vi "Update Measurement from Metadata.vi"(7 "client service_class":string, 8 "error in":errorcluster, 9 "default value":variant, 10 "metadata":T1, 11 "file refnums":refnum<vi>[](array[refnum])) -> (0 "error out":errorcluster)   [LabVIEW 2021, in "NI Measurement V2 Client Generator Runtime.lvlib"]
uses:
  NI Measurement V2 Client Generator Runtime.lvlib
  <vilib>/gRPC/Generated APIs/ni/measurementlink/measurement/v2/Measurement Service Client V2/RPC Messages/ni_measurementlink_measurement_v2_GetMetadataResponse.ctl
  <vilib>/gRPC/Generated APIs/ni/measurementlink/measurement/v2/Measurement Service Client V2/RPC Messages/ni_measurementlink_measurement_v2_MeasurementDetails.ctl
  <vilib>/gRPC/Generated APIs/ni/measurementlink/measurement/v2/Measurement Service Client V2/RPC Messages/ni_measurementlink_measurement_v2_MeasurementSignature.ctl
  <vilib>/gRPC/Generated APIs/ni/measurementlink/measurement/v2/Measurement Service Client V2/RPC Messages/ni_measurementlink_measurement_v2_ConfigurationParameter.ctl
  <vilib>/gRPC/Generated APIs/ni/measurementlink/measurement/v2/Measurement Service Client V2/RPC Messages/google_protobuf_Field_Kind.ctl
  <vilib>/gRPC/Generated APIs/ni/measurementlink/measurement/v2/Measurement Service Client V2/RPC Messages/ni_measurementlink_measurement_v2_ConfigurationParameter_AnnotationsEntry.ctl
  <vilib>/gRPC/Generated APIs/ni/measurementlink/measurement/v2/Measurement Service Client V2/RPC Messages/google_protobuf_Any.ctl
  <vilib>/gRPC/Generated APIs/ni/measurementlink/measurement/v2/Measurement Service Client V2/RPC Messages/ni_measurementlink_measurement_v2_Output.ctl
  <vilib>/gRPC/Generated APIs/ni/measurementlink/measurement/v2/Measurement Service Client V2/RPC Messages/ni_measurementlink_measurement_v2_Output_AnnotationsEntry.ctl
  <vilib>/gRPC/Generated APIs/ni/measurementlink/measurement/v2/Measurement Service Client V2/RPC Messages/ni_measurementlink_measurement_v2_UserInterfaceDetails.ctl
  <vilib>/Utility/traverseref.llb/TRef TravTarget.ctl
  Client Generator Error Strings Global.vi
  <vilib>/Utility/traverseref.llb/VI Scripting - Traverse.lvlib
  <vilib>/gRPC/Generated APIs/ni/measurementlink/measurement/v2/Measurement Service Client V2/Measurement Service Client V2.lvlib
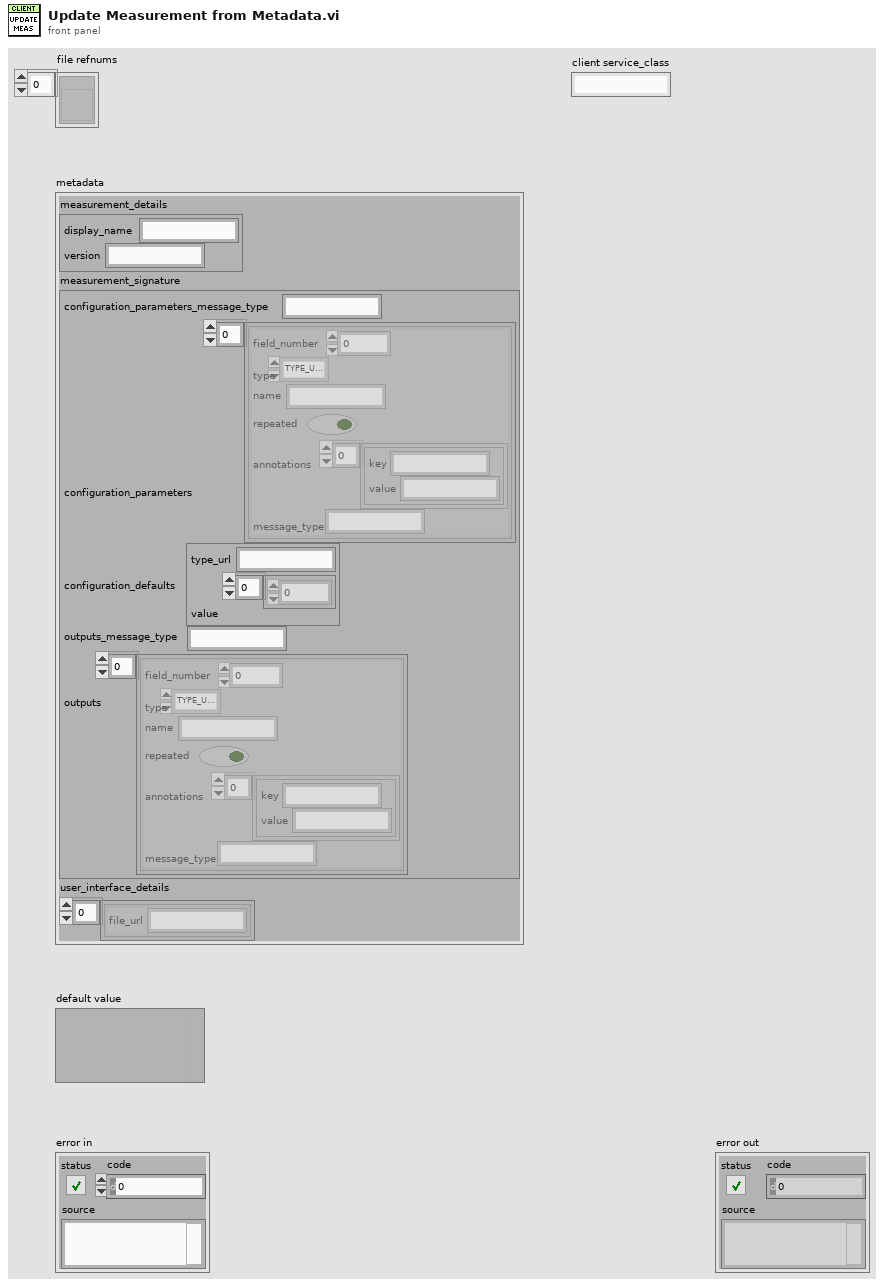
[diagram p1: front panel]
types:
  T1 = typedef "Measurement Service Client V2.lvlib/ni_measurementlink_measurement_v2_GetMetadataResponse.ctl" = cluster{"measurement_details":T2, "measurement_signature":T3, "user_interface_details":T10[]}
  T2 = typedef "Measurement Service Client V2.lvlib/ni_measurementlink_measurement_v2_MeasurementDetails.ctl" = cluster{"display_name":string, "version":string}
  T3 = typedef "Measurement Service Client V2.lvlib/ni_measurementlink_measurement_v2_MeasurementSignature.ctl" = cluster{"configuration_parameters_message_type":string, "configuration_parameters":T4[], "configuration_defaults":T7, "outputs_message_type":string, "outputs":T8[]}
  T4 = typedef "Measurement Service Client V2.lvlib/ni_measurementlink_measurement_v2_ConfigurationParameter.ctl" = cluster{"field_number":i32, "type":T5, "name":string, "repeated":bool, "annotations":T6[], "message_type":string}
  T5 = typedef "Measurement Service Client V2.lvlib/google_protobuf_Field_Kind.ctl" = enum32{"TYPE_UNKNOWN", "TYPE_DOUBLE", "TYPE_FLOAT", "TYPE_INT64", "TYPE_UINT64", "TYPE_INT32", "TYPE_FIXED64", "TYPE_FIXED32", "TYPE_BOOL", "TYPE_STRING", "TYPE_GROUP", "TYPE_MESSAGE", "TYPE_BYTES", "TYPE_UINT32", "TYPE_ENUM", "TYPE_SFIXED32", "TYPE_SFIXED64", "TYPE_SINT32", "TYPE_SINT64"}
  T6 = typedef "Measurement Service Client V2.lvlib/ni_measurementlink_measurement_v2_ConfigurationParameter_AnnotationsEntry.ctl" = cluster{"key":string, "value":string}
  T7 = typedef "Measurement Service Client V2.lvlib/google_protobuf_Any.ctl" = cluster{"type_url":string, "value":u8[]}
  T8 = typedef "Measurement Service Client V2.lvlib/ni_measurementlink_measurement_v2_Output.ctl" = cluster{"field_number":i32, "type":T5, "name":string, "repeated":bool, "annotations":T9[], "message_type":string}
  T9 = typedef "Measurement Service Client V2.lvlib/ni_measurementlink_measurement_v2_Output_AnnotationsEntry.ctl" = cluster{"key":string, "value":string}
  T10 = typedef "Measurement Service Client V2.lvlib/ni_measurementlink_measurement_v2_UserInterfaceDetails.ctl" = cluster{"file_url":string}
  T11 = typedef "TRef TravTarget.ctl" = enum16{"FP", "BD", "Other"}
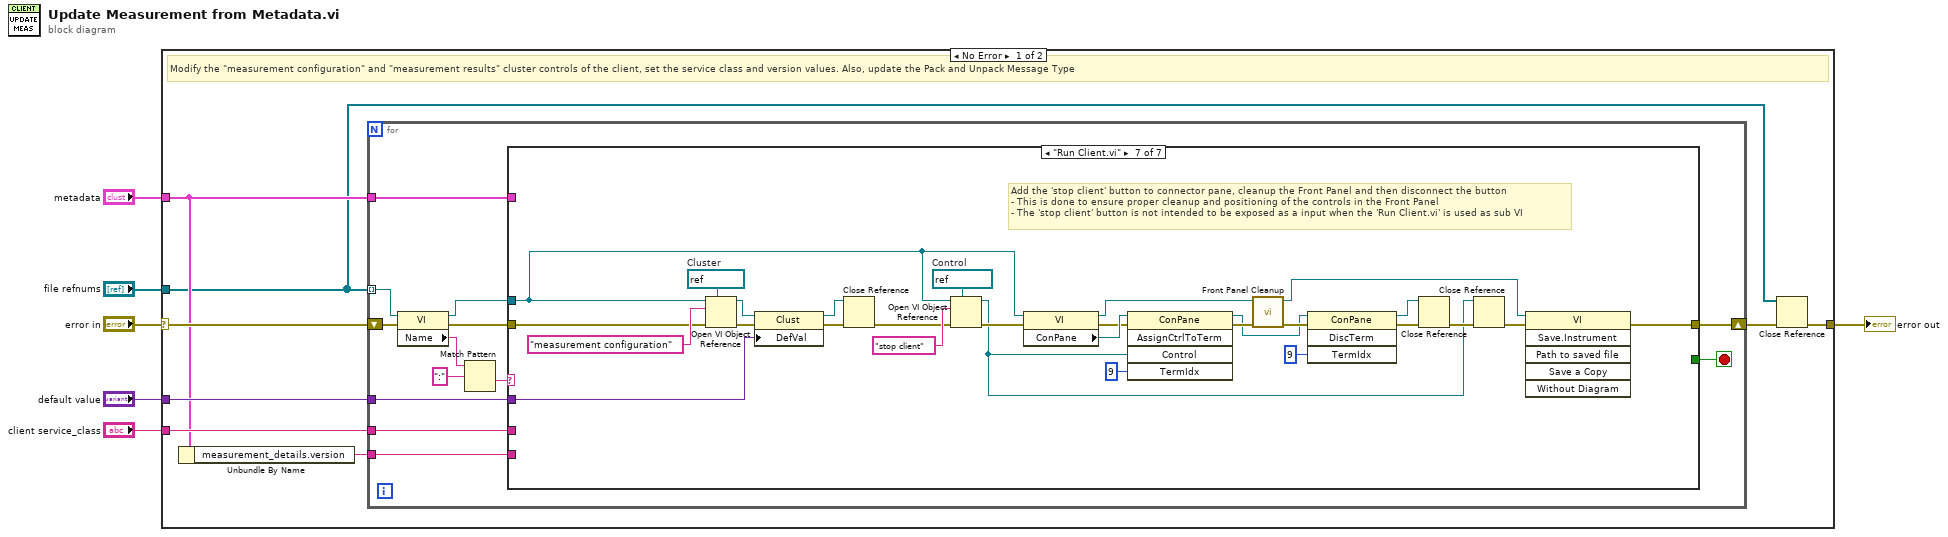
[diagram p0: block diagram]
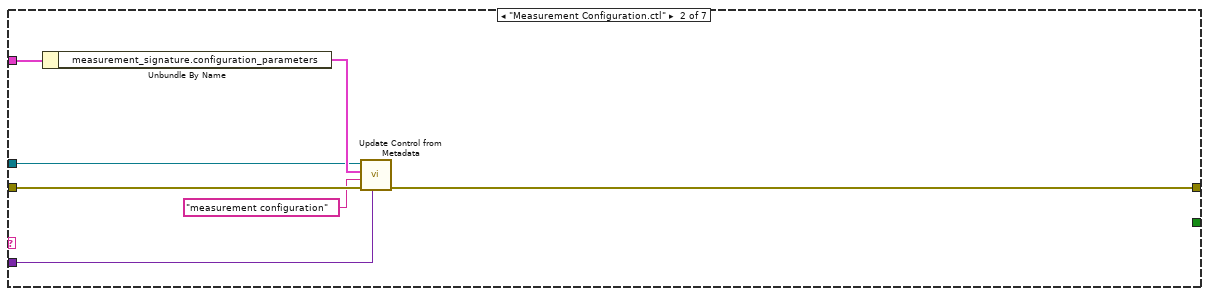
[diagram p3: hidden frame]
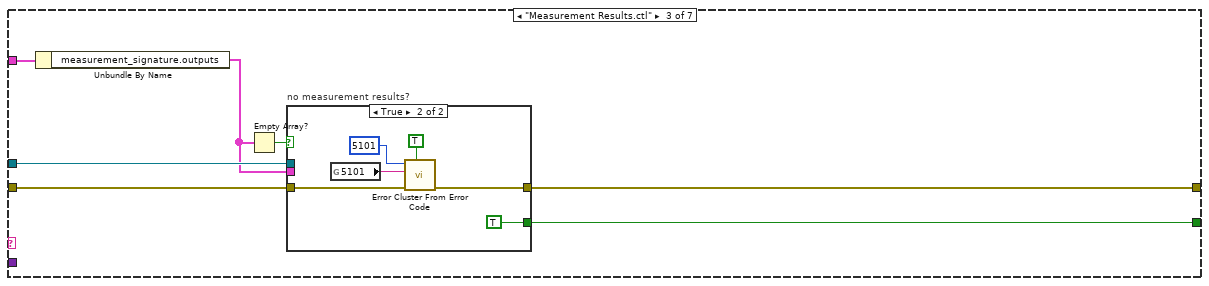
[diagram p4: hidden frame]
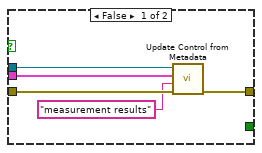
[diagram p5: hidden frame]
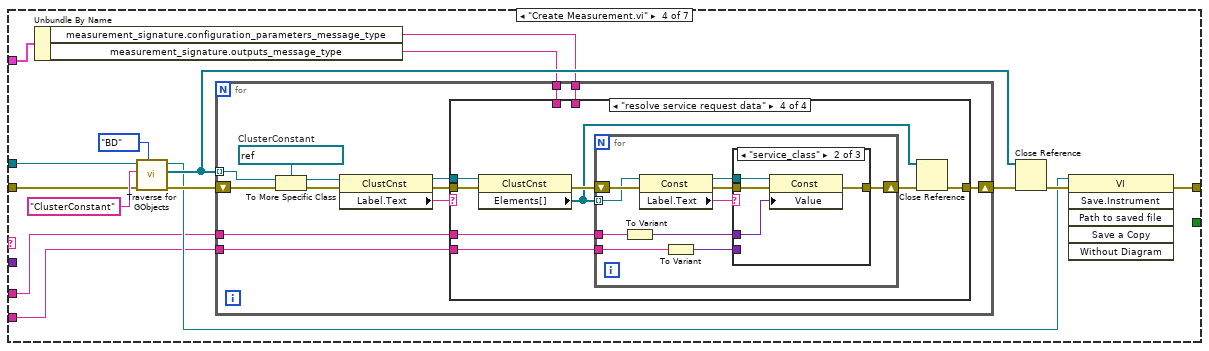
[diagram p6: hidden frame]
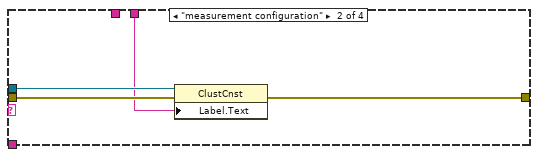
[diagram p8: hidden frame]
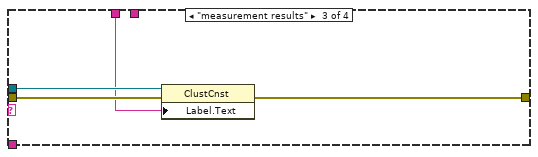
[diagram p9: hidden frame]
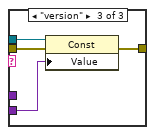
[diagram p11: hidden frame]
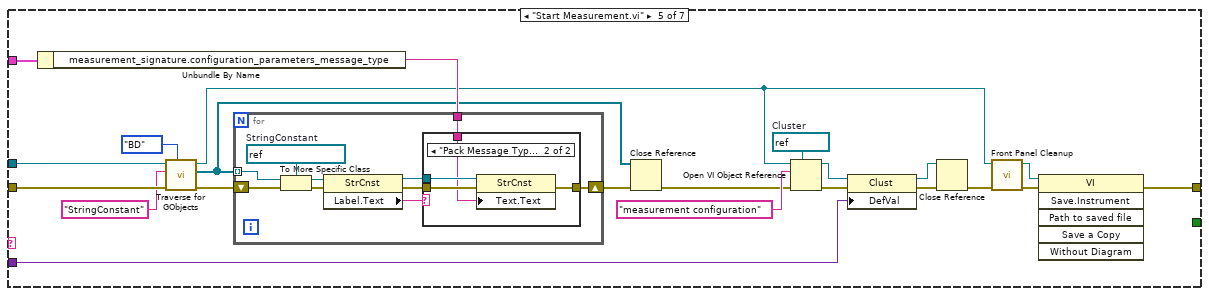
[diagram p12: hidden frame]
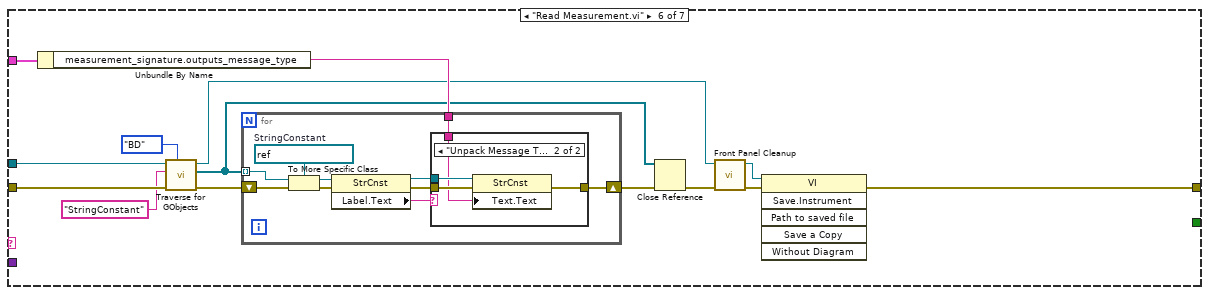
[diagram p14: hidden frame]
diagram:
  n1 = case shown="No Error" "error in" {
    selector: "error in" -> [w14 w212]
    tunnel: "client service_class" -> [w13 _]
    tunnel: "file refnums" -> [w7 _]
    tunnel: "default value" -> [w12 _]
    tunnel: "metadata" -> [w11 _]
    tunnel: [w8 w212] -> w1
    frame No Error {
      # "Modify the \"measurement configuration\" and \"measurement results\" cluster controls of the client, set the service class and version values. Also, update the Pack and Unpack Message Type"
      n2 = Unbundle By Name(w11) -> ("measurement_details.version"=w10:string)
      n3 = for {
        shift-right: [w26] -> w9
        shift-left: w14 -> [w27]
        tunnel: w7 -> [w24] mode=indexing
        tunnel: w13 -> [w21]
        tunnel: w12 -> [w20]
        tunnel: w11 -> [w19]
        tunnel: w10 -> [w18]
        stop <- w15 stop-if-true
        n4 = property class="VI"(reference=w24, error in=w27) -> (reference out=w16:refnum<vi>, error out=w25:errorcluster, "Name"=w22:string)
        n5 = Match Pattern(string=w22, regular expression=":") -> (after substring=w17:string)  [unwired: 1 in, 3 out]
        n6 = case shown="\"Run Client.vi\"" w17 {
          tunnel: w25 -> [w28 w35 w42 w60 w139 w168 w205]
          tunnel: [w28 w31 w40 w54 w120 w157 w190] -> w26
          tunnel: w16 -> [_ w32 w41 w61 w138 w167 w198]
          tunnel: w21 -> [_ _ _ w57 _ _ _]
          tunnel: w20 -> [_ w30 _ _ w128 _ w204]
          tunnel: w19 -> [_ w29 w39 w56 w123 w160 _]
          tunnel: w18 -> [_ _ _ w55 _ _ _]
          tunnel: [_ _ w36 _ _ _ _] -> w15
          frame Default {
          }
          frame "Measurement Configuration.ctl" {
            n7 = Unbundle By Name(w29) -> ("measurement_signature.configuration_parameters"=w33:T4[])
            n8 = call "Update Control from Metadata.vi"("default_value"=w30, "error in"=w35, "control name"="measurement configuration", "parameter data"=w33, "vi refnum"=w32) -> ("error out"=w31:errorcluster)  [unwired: 6 in]
          }
          frame "Measurement Results.ctl" {
            n9 = Unbundle By Name(w39) -> ("measurement_signature.outputs"=w38:T8[])
            n10 = Empty Array?(array=w38) -> (empty?=w37:bool)
            n11 = case "no measurement results?" shown="True" w37 {
              tunnel: w42 -> [w47 w50]
              tunnel: w38 -> [w45 _]
              tunnel: w41 -> [w44 _]
              tunnel: [w43 w49] -> w40
              tunnel: [_ TRUE] -> w36
              frame False {
                n12 = call "Update Control from Metadata.vi"("error in"=w47, "control name"="measurement results", "parameter data"=w45, "vi refnum"=w44) -> ("error out"=w43:errorcluster)  [unwired: 7 in]
              }
              frame True {
                n13 = global read "Client Generator Error Strings Global.vi" "5101"() -> (w52:string)
                n14 = call <vilib>:"Error Cluster From Error Code.vi"("show call chain? (False)"=TRUE, "error in (no error)"=w50, "error message (\"\")"=w52, "error code (0)"=5101) -> ("error out"=w49:errorcluster)  [unwired: 5 in]
              }
            }
          }
          frame "Create Measurement.vi" {
            n15 = Unbundle By Name(w56) -> ("measurement_signature.configuration_parameters_message_type"=w64:string, "measurement_signature.outputs_message_type"=w63:string)
            n16 = call <vilib>:"Traverse for GObjects.vi"("Traverse Target"=TRef_TravTarget."BD", "error in (no error)"=w60, "Class Name"="ClusterConstant", "VI Refnum"=w61) -> ("error out"=w68:errorcluster, "References"=w66:refnum<vi>[], "dup VI Refnum"=w58:refnum<vi>)  [unwired: 4 in, 1 out]
            n17 = for {
              shift-right: [w76] -> w62
              shift-left: w68 -> [w81]
              tunnel: w66 -> [w79] mode=indexing
              tunnel: w64 -> [w74]
              tunnel: w63 -> [w73]
              tunnel: w57 -> [w70]
              tunnel: w55 -> [w69]
              w72 = refnum<vi> refnum  # ClusterConstant
              n18 = To More Specific Class(target class=w72, reference=w79, error in=w81) -> (specific class reference=w78:refnum<vi>, error out=w80:errorcluster)
              n19 = property class="ClustCnst"(reference=w78, error in=w80) -> (reference out=w75:refnum<vi>, error out=w77:errorcluster, "Label.Text"=w71:string)
              n20 = case shown="\"resolve service request data\"" w71 {
                tunnel: [w82 w85 w89 w95] -> w76
                tunnel: w77 -> [w82 w86 w90 w98]
                tunnel: w75 -> [_ w84 w88 w97]
                tunnel: w74 -> [_ w83 _ _]
                tunnel: w73 -> [_ _ w87 _]
                tunnel: w70 -> [_ _ _ w93]
                tunnel: w69 -> [_ _ _ w92]
                frame Default {
                }
                frame "measurement configuration" {
                  n21 = property class="ClustCnst"(reference=w84, error in=w86, "Label.Text"=w83) -> (error out=w85:errorcluster)  [unwired: 1 out]
                }
                frame "measurement results" {
                  n22 = property class="ClustCnst"(reference=w88, error in=w90, "Label.Text"=w87) -> (error out=w89:errorcluster)  [unwired: 1 out]
                }
                frame "resolve service request data" {
                  n23 = property class="ClustCnst"(reference=w97, error in=w98) -> (error out=w96:errorcluster, "Elements[]"=w94:refnum<vi>[])  [unwired: 1 out]
                  n24 = for {
                    tunnel: w94 -> [w107] mode=indexing
                    tunnel: w93 -> [w101]
                    tunnel: w92 -> [w100]
                    shift-right: [w99] -> w91
                    shift-left: w96 -> [w108]
                    n25 = To Variant(anything=w101) -> (Variant=w102:variant)
                    n26 = property class="Const"(reference=w107, error in=w108) -> (reference out=w104:refnum<vi>, error out=w105:errorcluster, "Label.Text"=w106:string)
                    n27 = To Variant(anything=w100) -> (Variant=w103:variant)
                    n28 = case shown="\"service_class\"" w106 {
                      tunnel: w105 -> [w109 w113 w117]
                      tunnel: w104 -> [_ w112 w116]
                      tunnel: [w109 w111 w115] -> w99
                      tunnel: w103 -> [_ _ w114]
                      tunnel: w102 -> [_ w110 _]
                      frame Default {
                      }
                      frame "service_class" {
                        n29 = property class="Const"(reference=w112, error in=w113, "Value"=w110) -> (error out=w111:errorcluster)  [unwired: 1 out]
                      }
                      frame "version" {
                        n30 = property class="Const"(reference=w116, error in=w117, "Value"=w114) -> (error out=w115:errorcluster)  [unwired: 1 out]
                      }
                    }
                  }
                  n31 = Close Reference(reference=w94, error in (no error)=w91) -> (error out=w95:errorcluster)
                }
              }
            }
            n32 = Close Reference(reference=w66, error in (no error)=w62) -> (error out=w59:errorcluster)
            n33 = invoke class="VI" method="Save.Instrument"(reference=w58, error in=w59) -> (error out=w54:errorcluster)  [unwired: 4 in, 5 out]
          }
          frame "Start Measurement.vi" {
            w131 = refnum<vi> refnum  # Cluster
            n34 = Unbundle By Name(w123) -> ("measurement_signature.configuration_parameters_message_type"=w134:string)
            n35 = call <vilib>:"Traverse for GObjects.vi"("Traverse Target"=TRef_TravTarget."BD", "error in (no error)"=w139, "Class Name"="StringConstant", "VI Refnum"=w138) -> ("error out"=w135:errorcluster, "References"=w124:refnum<vi>[], "dup VI Refnum"=w119:refnum<vi>)  [unwired: 4 in, 1 out]
            n36 = for {
              shift-right: [w149] -> w133
              shift-left: w135 -> [w148]
              tunnel: w124 -> [w146] mode=indexing
              tunnel: w134 -> [w140]
              w145 = refnum<vi> refnum  # StringConstant
              n37 = To More Specific Class(target class=w145, reference=w146, error in=w148) -> (specific class reference=w143:refnum<vi>, error out=w147:errorcluster)
              n38 = property class="StrCnst"(reference=w143, error in=w147) -> (reference out=w142:refnum<vi>, error out=w144:errorcluster, "Label.Text"=w141:string)
              n39 = case shown="\"Pack Message Type\"" w141 {
                tunnel: [w150 w154] -> w149
                tunnel: w144 -> [w150 w153]
                tunnel: w142 -> [_ w152]
                tunnel: w140 -> [_ w151]
                frame Default {
                }
                frame "Pack Message Type" {
                  n40 = property class="StrCnst"(reference=w152, error in=w153, "Text.Text"=w151) -> (error out=w154:errorcluster)  [unwired: 1 out]
                }
              }
            }
            n41 = Close Reference(reference=w124, error in (no error)=w133) -> (error out=w125:errorcluster)
            n42 = Open VI Object Reference(7:w131, 8:w125, 10:"measurement configuration" ("name/order"), 11:w119) -> (0:w132:errorcluster, 3:w129:refnum<vi>)
            n43 = property class="Clust"(reference=w129, error in=w132, "DefVal"=w128) -> (reference out=w127:refnum<vi>, error out=w130:errorcluster)
            n44 = Close Reference(reference=w127, error in (no error)=w130) -> (error out=w118:errorcluster)
            n45 = call "Front Panel Cleanup.vi"("error in"=w118, "vi refnum"=w119) -> ("error out"=w121:errorcluster, "vi refnum out"=w122:refnum<vi>)  [unwired: 8 in]
            n46 = invoke class="VI" method="Save.Instrument"(reference=w122, error in=w121) -> (error out=w120:errorcluster)  [unwired: 4 in, 5 out]
          }
          frame "Read Measurement.vi" {
            n47 = Unbundle By Name(w160) -> ("measurement_signature.outputs_message_type"=w163:string)
            n48 = call <vilib>:"Traverse for GObjects.vi"("Traverse Target"=TRef_TravTarget."BD", "error in (no error)"=w168, "Class Name"="StringConstant", "VI Refnum"=w167) -> ("error out"=w164:errorcluster, "References"=w161:refnum<vi>[], "dup VI Refnum"=w155:refnum<vi>)  [unwired: 4 in, 1 out]
            n49 = for {
              shift-right: [w169] -> w162
              shift-left: w164 -> [w178]
              tunnel: w161 -> [w176] mode=indexing
              tunnel: w163 -> [w170]
              w175 = refnum<vi> refnum  # StringConstant
              n50 = To More Specific Class(target class=w175, reference=w176, error in=w178) -> (specific class reference=w173:refnum<vi>, error out=w177:errorcluster)
              n51 = property class="StrCnst"(reference=w173, error in=w177) -> (reference out=w172:refnum<vi>, error out=w174:errorcluster, "Label.Text"=w171:string)
              n52 = case shown="\"Unpack Message Type\"" w171 {
                tunnel: [w179 w183] -> w169
                tunnel: w174 -> [w179 w182]
                tunnel: w172 -> [_ w181]
                tunnel: w170 -> [_ w180]
                frame Default {
                }
                frame "Unpack Message Type" {
                  n53 = property class="StrCnst"(reference=w181, error in=w182, "Text.Text"=w180) -> (error out=w183:errorcluster)  [unwired: 1 out]
                }
              }
            }
            n54 = Close Reference(reference=w161, error in (no error)=w162) -> (error out=w156:errorcluster)
            n55 = call "Front Panel Cleanup.vi"("error in"=w156, "vi refnum"=w155) -> ("error out"=w158:errorcluster, "vi refnum out"=w159:refnum<vi>)  [unwired: 8 in]
            n56 = invoke class="VI" method="Save.Instrument"(reference=w159, error in=w158) -> (error out=w157:errorcluster)  [unwired: 4 in, 5 out]
          }
          frame "Run Client.vi" {
            w187 = refnum<vi> refnum  # Control
            w210 = refnum<vi> refnum  # Cluster
            # "Add the 'stop client' button to connector pane, cleanup the Front Panel and then disconnect the button\n- This is done to ensure proper cleanup and positioning of the controls in the Front Panel\n- The 'stop client' button is not intended to be exposed as a input when the 'Run Client.vi' is used as sub VI"
            n57 = Open VI Object Reference(7:w210, 8:w205, 10:"measurement configuration" ("name/order"), 11:w198) -> (0:w211:errorcluster, 3:w208:refnum<vi>)
            n58 = property class="Clust"(reference=w208, error in=w211, "DefVal"=w204) -> (reference out=w207:refnum<vi>, error out=w209:errorcluster)
            n59 = Close Reference(reference=w207, error in (no error)=w209) -> (error out=w199:errorcluster)
            n60 = Open VI Object Reference(7:w187, 8:w199, 10:"stop client" ("name/order"), 11:w198) -> (0:w200:errorcluster, 3:w185:refnum<vi>)
            n61 = property class="VI"(reference=w198, error in=w200) -> (reference out=w197:refnum<vi>, error out=w201:errorcluster, "ConPane"=w202:refnum<vi>)
            n62 = invoke class="ConPane" method="AssignCtrlToTerm"(reference=w202, error in=w201, "Control"=w185, "TermIdx"=u32 9 ("Terminal Index")) -> (reference out=w194:refnum<vi>, error out=w196:errorcluster)  [unwired: 1 in, 3 out]
            n63 = call "Front Panel Cleanup.vi"("error in"=w196, "vi refnum"=w197) -> ("error out"=w195:errorcluster, "vi refnum out"=w191:refnum<vi>)  [unwired: 8 in]
            n64 = invoke class="ConPane" method="DiscTerm"(reference=w194, error in=w195, "TermIdx"=u32 9 ("Terminal Index")) -> (reference out=w184:refnum<vi>, error out=w193:errorcluster)  [unwired: 1 in, 2 out]
            n65 = Close Reference(reference=w184, error in (no error)=w193) -> (error out=w192:errorcluster)
            n66 = Close Reference(reference=w185, error in (no error)=w192) -> (error out=w186:errorcluster)
            n67 = invoke class="VI" method="Save.Instrument"(reference=w191, error in=w186) -> (error out=w190:errorcluster)  [unwired: 4 in, 5 out]
          }
        }
      }
      n68 = Close Reference(reference=w7, error in (no error)=w9) -> (error out=w8:errorcluster)
    }
    frame Error {
      # "Pass"
    }
  }
  "error out" <- w1
